vi "Initialize Interfaces for Runner.vi"(8 "error in":errorcluster, 11 "Logger Enqueuer":refnum<class "Message Enqueuer.lvclass">) -> (0 "error out":errorcluster, 3 "Interfaces":T1)   [LabVIEW 2026]
doc: "This VI initializes all required interfaces for the Runner and sets the logger enqueuer where needed."
uses:
  Classes/Hash Whitelist Handler/Hash Whitelist Handler.lvclass
  C:/Users/juanj/Documents/hasbun_wood_engineering/github/py2vi/labview/Classes/Hash Whitelist Handler/Hash Whitelist Handler.lvclass
  C:/Users/juanj/Documents/hasbun_wood_engineering/github/py2vi/labview/Interfaces/IHash Whitelist Handler/IHash Whitelist Handler.lvclass
  C:/Users/juanj/Documents/hasbun_wood_engineering/github/py2vi/labview/Interfaces/ILogger Client/ILogger Client/ILogger Client.lvclass
  Classes/Project Manager/Project Manager.lvclass
  C:/Users/juanj/Documents/hasbun_wood_engineering/github/py2vi/labview/Classes/Project Manager/Project Manager.lvclass
  C:/Users/juanj/Documents/hasbun_wood_engineering/github/py2vi/labview/Interfaces/IProject Manager/IProject Manager.lvclass
  Classes/File Manager/File Manager.lvclass
  C:/Users/juanj/Documents/hasbun_wood_engineering/github/py2vi/labview/Classes/File Manager/File Manager.lvclass
  C:/Users/juanj/Documents/hasbun_wood_engineering/github/py2vi/labview/Interfaces/IFile Manager/IFile Manager.lvclass
  Classes/Python Caller/Python Caller.lvclass
  C:/Users/juanj/Documents/hasbun_wood_engineering/github/py2vi/labview/Classes/Python Caller/Python Caller.lvclass
  C:/Users/juanj/Documents/hasbun_wood_engineering/github/py2vi/labview/Interfaces/IPython Caller/IPython Caller.lvclass
  Classes/Element Manager/Element Manager.lvclass
  C:/Users/juanj/Documents/hasbun_wood_engineering/github/py2vi/labview/Classes/Element Manager/Element Manager.lvclass
  C:/Users/juanj/Documents/hasbun_wood_engineering/github/py2vi/labview/Interfaces/IElement Manager/IElement Manager.lvclass
  Classes/LV File Creator/LV File Creator.lvclass
  C:/Users/juanj/Documents/hasbun_wood_engineering/github/py2vi/labview/Classes/LV File Creator/LV File Creator.lvclass
  C:/Users/juanj/Documents/hasbun_wood_engineering/github/py2vi/labview/Interfaces/ILV File Creator/ILV File Creator.lvclass
  Interfaces/IHash Whitelist Handler/IHash Whitelist Handler.lvclass
  Interfaces/ILV File Creator/ILV File Creator.lvclass
  Interfaces/IElement Manager/IElement Manager.lvclass
  Interfaces/IPython Caller/IPython Caller.lvclass
  Interfaces/IFile Manager/IFile Manager.lvclass
  Interfaces/IProject Manager/IProject Manager.lvclass
  Interfaces/IRunner/IRunner/Interfaces--cluster.ctl
  Interfaces/IRunner/IRunner/IRunner.lvclass
  <vilib>/ActorFramework/Message Enqueuer/Message Enqueuer.lvclass
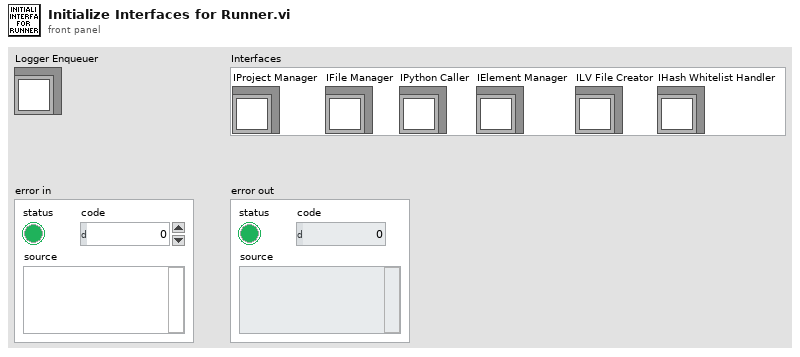
[diagram p1: front panel]
types:
  T1 = typedef "IRunner.lvlib/IRunner.lvclass/Interfaces--cluster.ctl" = cluster{"IProject Manager":refnum<class "IProject Manager.lvclass">, "IFile Manager":refnum<class "IFile Manager.lvclass">, "IPython Caller":refnum<class "IPython Caller.lvclass">, "IElement Manager":refnum<class "IElement Manager.lvclass">, "ILV File Creator":refnum<class "ILV File Creator.lvclass">, "IHash Whitelist Handler":refnum<class "IHash Whitelist Handler.lvclass">}
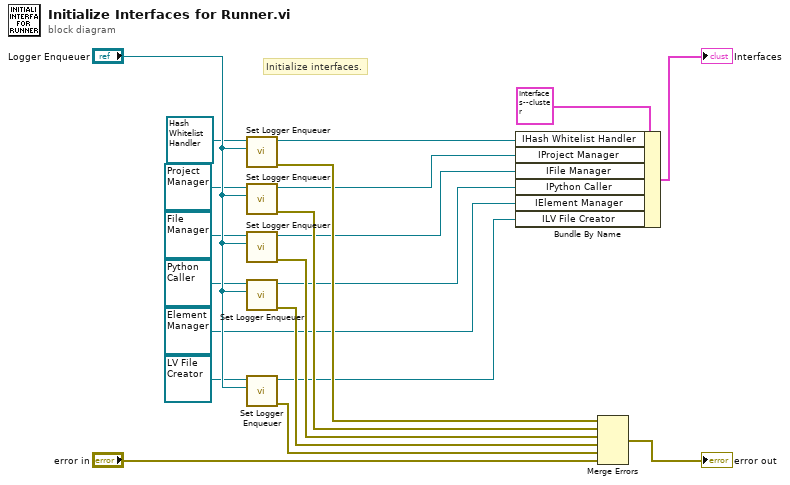
[diagram p0: block diagram]
diagram:
  # "Initialize interfaces."
  n1 = call-dynamic "Set Logger Enqueuer.vi"("Logger"="Logger Enqueuer", "Hash Whitelist Handler in"=refnum<class "Hash Whitelist Handler.lvclass"> refnum ("Hash Whitelist Handler.lvclass")) -> ("error out"=w21:errorcluster, "Hash Whitelist Handler out"=w13:refnum<class "Hash Whitelist Handler.lvclass">)  [unwired: 8 in]
  n2 = call-dynamic "Set Logger Enqueuer.vi"("Logger"="Logger Enqueuer", "Project Manager in"=refnum<class "Project Manager.lvclass"> refnum ("Project Manager.lvclass")) -> ("error out"=w15:errorcluster, "Project Manager out"=w4:refnum<class "Project Manager.lvclass">)  [unwired: 8 in]
  n3 = call-dynamic "Set Logger Enqueuer.vi"("Logger"="Logger Enqueuer", "File Manager in"=refnum<class "File Manager.lvclass"> refnum ("File Manager.lvclass")) -> ("error out"=w16:errorcluster, "File Manager out"=w5:refnum<class "File Manager.lvclass">)  [unwired: 8 in]
  n4 = call-dynamic "Set Logger Enqueuer.vi"("Logger"="Logger Enqueuer", "Python Caller in"=refnum<class "Python Caller.lvclass"> refnum ("Python Caller.lvclass")) -> ("error out"=w17:errorcluster, "Python Caller out"=w7:refnum<class "Python Caller.lvclass">)  [unwired: 8 in]
  n5 = call-dynamic "Set Logger Enqueuer.vi"("Logger"="Logger Enqueuer", "LV File Creator in"=refnum<class "LV File Creator.lvclass"> refnum ("LV File Creator.lvclass")) -> ("error out"=w18:errorcluster, "LV File Creator out"=w10:refnum<class "LV File Creator.lvclass">)  [unwired: 8 in]
  n6 = Bundle By Name(cluster=T1 {"IProject Manager"=refnum, "IFile Manager"=refnum, "IPython Caller"=refnum, "IElement Manager"=refnum, "ILV File Creator"=refnum, "IHash Whitelist Handler"=refnum} ("Interfaces"), "IHash Whitelist Handler"=w13, "IProject Manager"=w4, "IFile Manager"=w5, "IPython Caller"=w7, "IElement Manager"=refnum<class "Element Manager.lvclass"> refnum ("Element Manager.lvclass"), "ILV File Creator"=w10) -> (→"Interfaces":T1)
  n7 = Merge Errors(w21, w15, w16, w17, w18, "error in") -> (→"error out":errorcluster)
